vi "Read Value.vi"(8 "error in (no error)":errorcluster, 11 "NT Scalar in":refnum<class "NT Scalar.lvclass">) -> (0 "error out":errorcluster, 2 "value":variant, 3 "NT Scalar out":refnum<class "NT Scalar.lvclass">)   [LabVIEW 2020, in "PV Access.lvlib" / "PV Data.lvlib" / "NT Scalar.lvclass"]
uses:
  NT Scalar.lvclass
  NT Scalar.lvclass/NT Scalar.ctl
  3c5cef72-99eb-4319-ac6c-76cddedc9ff7.vi
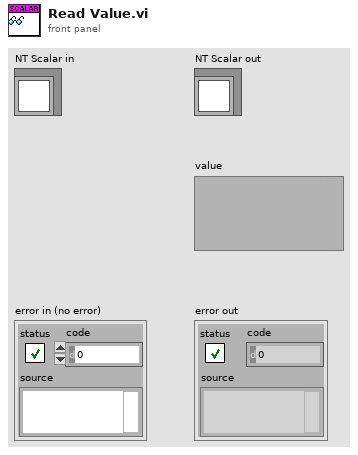
[diagram p1: front panel]
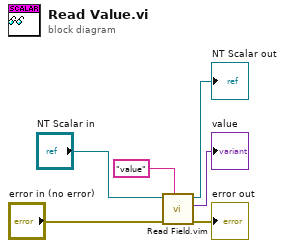
[diagram p0: block diagram]
diagram:
  n1 = call "Read Field.vim"("field"="value", "error in"="error in (no error)", "Base Interface in"="NT Scalar in") -> ("error out"=→"error out":errorcluster, "value"=→"value":variant, "Base Interface out"=→"NT Scalar out":refnum<class "NT Scalar.lvclass">)  [unwired: 6 in]
